vi "get channel keys.vi"(11 "data allocations":T4) -> (0 "Output Map":T1[](array[typedef]), 1 "Input Map":T1[](array[typedef]), 2 "output subquery":string, 3 "input pk list":string[](array[string]))   [LabVIEW 2014, in "SQLite runtime.lvclass"]
uses:
  SQLite runtime.lvclass
  <vilib>/NI/Tag Bus Module Framework/channel/data tables.ctl
  <vilib>/NI/Tag Bus/dictionary/data dictionary.lvclass
  <vilib>/NI/Tag Bus/dictionary table pair.ctl
  <vilib>/NI/Tag Bus/table/data table.ctl
  data map.ctl
  <vilib>/NI/Tag Bus/tag/Data Type.ctl
  sqlite type.ctl
  <vilib>/NI/Tag Bus/table/data table.lvlib
  <vilib>/NI/Tag Bus/tag bus.lvlib
  <vilib>/NI/Tag Bus Module Framework/channel/TBM channel.lvclass
  <vilib>/NI/Tag Bus/tag/tag descriptor.lvclass
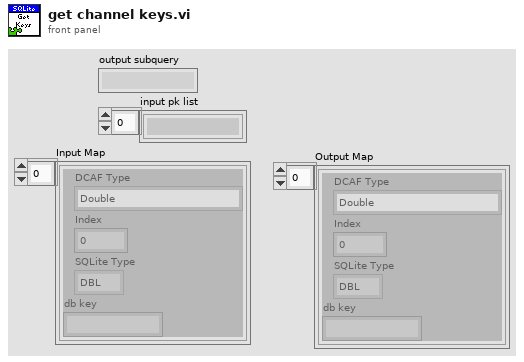
[diagram p1: front panel]
types:
  T1 = typedef "SQLite runtime.lvclass/data map.ctl" = cluster{"DCAF Type":T2, "Index":i32, "SQLite Type":T3, "db key":string}
  T2 = typedef "tag bus.lvlib/tag descriptor.lvclass/Data Type.ctl" = enum16{"Double", "Single", "I64", "I32", "I16", "I8", "U64", "U32", "U16", "U8", "Boolean", "String", "Array of Double", "Array of Single", "Array of I64", "Array of I32", "Array of I16", "Array of I8", "Array of U64", "Array of U32", "Array of U16", "Array of U8", "Array of Boolean", "Array of String"}
  T3 = typedef "SQLite runtime.lvclass/sqlite type.ctl" = enum16{"DBL", "I64", "String"}
  T4 = typedef "TBM channel.lvclass/data tables.ctl" = cluster{"input data":T5, "processing parameter":T5, "processing result":T5, "output data":T5}
  T5 = typedef "tag bus.lvlib/dictionary table pair.ctl" = cluster{"data dictionary":refnum<class "data dictionary.lvclass">, "data table":T6}
  T6 = typedef "tag bus.lvlib/data table.lvlib/data table.ctl" = cluster{"Double":dbl[], "Single":sgl[], "I64":i64[], "I32":i32[], "I16":i16[], "I8":i8[], "U64":u64[], "U32":u32[], "U16":u16[], "U8":u8[], "Boolean":bool[], "String":string[], "Array of Double":cluster{"DBL Array":dbl[]}[], "Array of Single":cluster{"SGL Array":sgl[]}[], "Array of I64":cluster{"I64 Array":i64[]}[], "Array of I32":cluster{"I32 Array":i32[]}[], "Array of I16":cluster{"I16 Array":i16[]}[], "Array of I8":cluster{"I8 Array":i8[]}[], "Array of U64":cluster{"U64 Array":u64[]}[], "Array of U32":cluster{"U32 Array":u32[]}[], "Array of U16":cluster{"U16 Array":u16[]}[], "Array of U8":cluster{"U8 Array":u8[]}[], "Array of Boolean":cluster{"Boolean Array":bool[]}[], "Array of String":cluster{"String Array":string[]}[]}
  T7 = typedef "tag bus.lvlib/data dictionary.lvclass/full data dictionary.ctl" = cluster{"Double":string[], "Single":string[], "I64":string[], "I32":string[], "I16":string[], "I8":string[], "U64":string[], "U32":string[], "U16":string[], "U8":string[], "Boolean":string[], "String":string[], "Array of Double":string[], "Array of Single":string[], "Array of I64":string[], "Array of I32":string[], "Array of I16":string[], "Array of I8":string[], "Array of U64":string[], "Array of U32":string[], "Array of U16":string[], "Array of U8":string[], "Array of Boolean":string[], "Array of String":string[]}
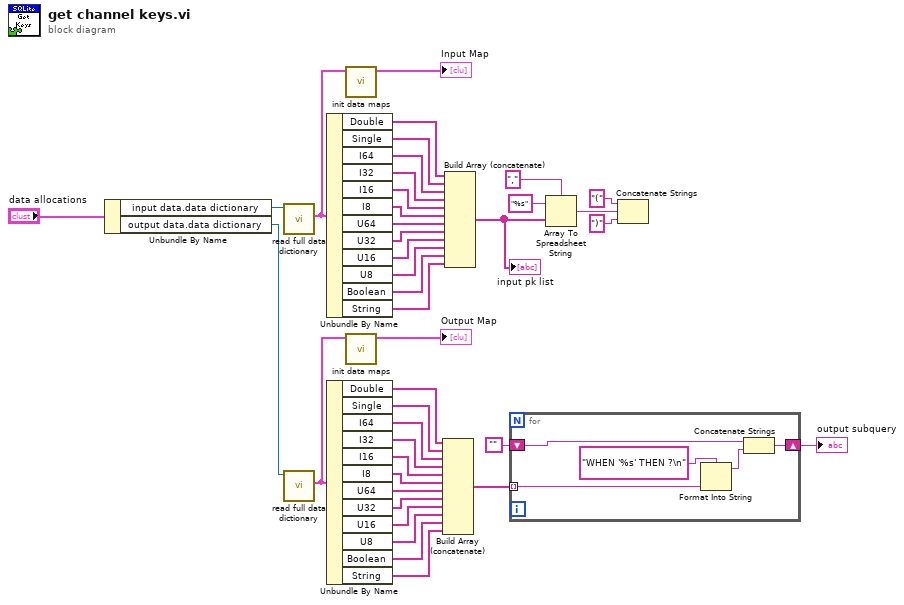
[diagram p0: block diagram]
diagram:
  n1 = Unbundle By Name("data allocations") -> ("input data.data dictionary"=w39:refnum<class "data dictionary.lvclass">, "output data.data dictionary"=w10:refnum<class "data dictionary.lvclass">)
  n2 = call <vilib>:"read full data dictionary.vi"("data dictionary in"=w39) -> ("dictionary"=w3:T7)  [unwired: 8 in, 2 out]
  n3 = call <vilib>:"read full data dictionary.vi"("data dictionary in"=w10) -> ("dictionary"=w5:T7)  [unwired: 8 in, 2 out]
  n4 = Unbundle By Name(w3) -> ("Double"=w38:string[], "Single"=w37:string[], "I64"=w36:string[], "I32"=w35:string[], "I16"=w34:string[], "I8"=w33:string[], "U64"=w32:string[], "U32"=w31:string[], "U16"=w30:string[], "U8"=w29:string[], "Boolean"=w28:string[], "String"=w27:string[])
  n5 = Unbundle By Name(w5) -> ("Double"=w1:string[], "Single"=w21:string[], "I64"=w20:string[], "I32"=w19:string[], "I16"=w18:string[], "I8"=w17:string[], "U64"=w16:string[], "U32"=w15:string[], "U16"=w14:string[], "U8"=w13:string[], "Boolean"=w12:string[], "String"=w11:string[])
  n6 = call "init data maps.vi"("input cluster"=w3) -> ("Data Maps Out"=→"Input Map":T1[])  [unwired: 10 in]
  n7 = call "init data maps.vi"("input cluster"=w5) -> ("Data Maps Out"=→"Output Map":T1[])  [unwired: 10 in]
  n8 = Build Array (concatenate)(w1, w21, w20, w19, w18, w17, w16, w15, w14, w13, w12, w11) -> (w9:string[])
  n9 = Build Array (concatenate)(w38, w37, w36, w35, w34, w33, w32, w31, w30, w29, w28, w27) -> (w6:string[])
  "input pk list" <- w6
  n10 = for {
    tunnel: w9 -> [w44] mode=indexing
    shift-right: [w43] -> w7
    shift-left: "" -> [w42]
    n11 = Format Into String(format string="WHEN '%s' THEN ?\n", w44) -> (resulting string=w41:string)  [unwired: 2 in, 1 out]
    n12 = Concatenate Strings(w42, w41) -> (w43:string)
  }
  "output subquery" <- w7
  n13 = Array To Spreadsheet String(delimiter (Tab)=",", array=w6, 3:"%s" ("format string")) -> (spreadsheet string=w24:string)
  n14 = Concatenate Strings("(" ("string"), w24, ")" ("string")) -> ()  [unwired: 1 out]
